vi "RFH-utility-split_low_data.vi"(7 "Frequency":dbl=1000000000.0, 11 "Common Format":T1) -> (2 "After":T1)   [LabVIEW 2020, in "RFH-Reflection_File_Handler.lvlib"]
doc: "Removes the data below a frequency from a Common Format cluster and returns the rest."
uses:
  RFH-Reflection_File_Handler.lvlib
  RFH-common_data_format.ctl
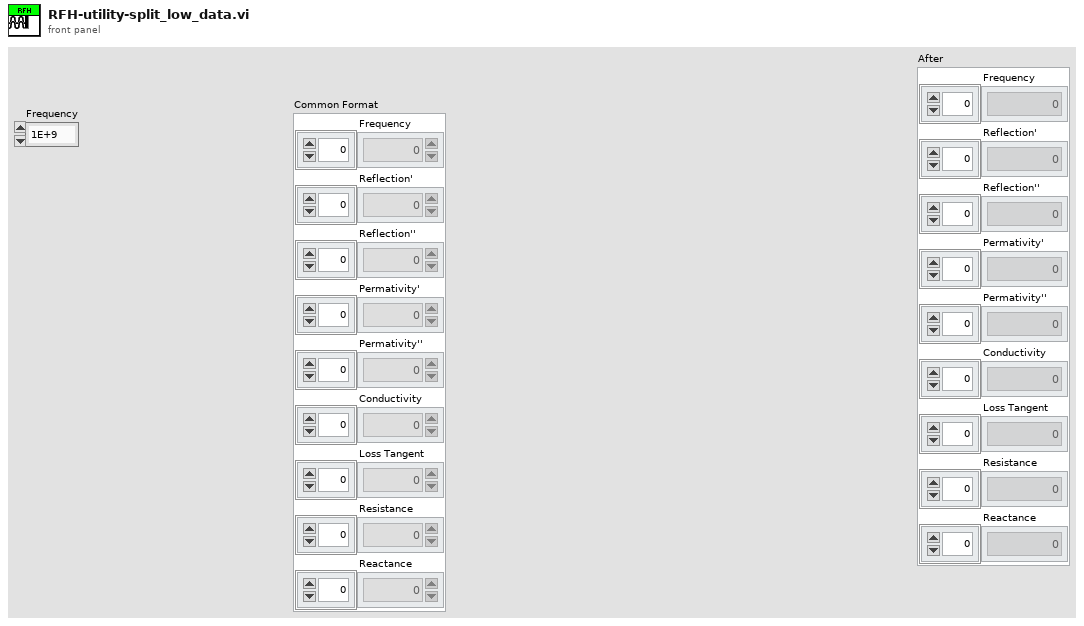
[diagram p1: front panel]
types:
  T1 = typedef "RFH-Reflection_File_Handler.lvlib/RFH-common_data_format.ctl" = cluster{"Frequency":dbl[], "Reflection'":dbl[], "Reflection''":dbl[], "Permativity'":dbl[], "Permativity''":dbl[], "Conductivity":dbl[], "Loss Tangent":dbl[], "Resistance":dbl[], "Reactance":dbl[]}
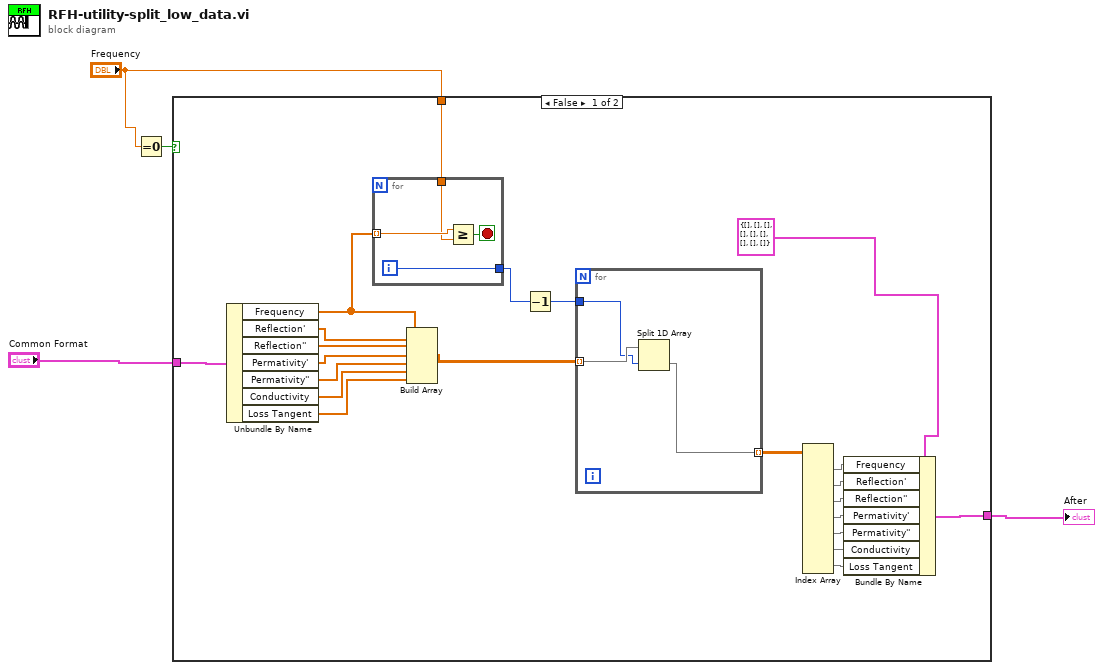
[diagram p0: block diagram]
diagram:
  n1 = Equal To 0?(x="Frequency") -> (x = 0?=w1:bool)
  n2 = case shown="False" w1 {
    tunnel: "Common Format" -> [w26 w34]
    tunnel: "Frequency" -> [w18 _]
    tunnel: [w6 w34] -> w3
    frame False {
      n3 = Unbundle By Name(w26) -> ("Frequency"=w19:dbl[], "Reflection'"=w25:dbl[], "Reflection''"=w24:dbl[], "Permativity'"=w23:dbl[], "Permativity''"=w22:dbl[], "Conductivity"=w21:dbl[], "Loss Tangent"=w20:dbl[])
      n4 = for {
        tunnel: w19 -> [w33] mode=indexing
        tunnel: w18 -> [w32]
        tunnel: [w30] -> w17
        i -> [w30]
        stop <- w31 stop-if-true
        n5 = Greater Or Equal?(x=w33, y=w32) -> (x >= y?=w31:bool)
      }
      n6 = Build Array(w19, w25, w24, w23, w22, w21, w20) -> (w16:dbl[][])
      n7 = Decrement(x=w17) -> (x-1=w5:i32)
      n8 = for {
        tunnel: w5 -> [w28]
        tunnel: w16 -> [w29] mode=indexing
        tunnel: [w27] -> w8 mode=indexing
        n9 = Split 1D Array(array=w29, index=w28) -> (second subarray=w27:dbl[])  [unwired: 1 out]
      }
      n10 = Index Array(array=w8) -> (element #1=w9:dbl[], element #2=w10:dbl[], element #3=w11:dbl[], element #4=w12:dbl[], element #5=w13:dbl[], element #6=w14:dbl[], element #7=w15:dbl[])  [unwired: 14 in]
      n11 = Bundle By Name(cluster=T1 {"Frequency"=[], "Reflection'"=[], "Reflection''"=[], "Permativity'"=[], "Permativity''"=[], "Conductivity"=[], "Loss Tangent"=[], "Resistance"=[], "Reactance"=[]} ("Common Format"), "Frequency"=w9, "Reflection'"=w10, "Reflection''"=w11, "Permativity'"=w12, "Permativity''"=w13, "Conductivity"=w14, "Loss Tangent"=w15) -> (w6:T1)
    }
    frame True {
    }
  }
  "After" <- w3
